vi "Cascade Config.vi"() -> (2 "FeedForward Constants Out":cluster{"kA":dbl, "kS":dbl, "kG":dbl, "kV":dbl}={"kA"=0.0, "kS"=0.0, "kG"=-0.25, "kV"=0.0}, 3 "Cascade Setpoints Config Out (Sensor Positions)":T2={"Array"=[{"Preset Name"=enum."Idle/Ground", "Cascade Pos"=0.0}, {"Preset Name"=enum."Raised L1", "Cascade Pos"=-3.112302245200002}, {"Preset Name"=enum."L2", "Cascade Pos"=-8.9212319508}, {"Preset Name"=enum."L2 Tip", "Cascade Pos"=-14.937623431600002}, {"Preset Name"=enum."L3", "Cascade Pos"=-21.991323788400003}, {"Preset Name"=enum."L3 Tip", "Cascade Pos"=-23.65101799}, {"Preset Name"=enum."Feeder", "Cascade Pos"=-16.4935867456}, {"Preset Name"=enum."\"Default\"", "Cascade Pos"=0.0}]})   [LabVIEW 2027]
uses:
  Cascade Positions.ctl
panel:
  in  "Cascade Setpoints Config (Sensor Pos)":T2={"Array"=[{"Preset Name"=enum."Idle/Ground", "Cascade Pos"=0.0}, {"Preset Name"=enum."Raised L1", "Cascade Pos"=8.0}, {"Preset Name"=enum."L2", "Cascade Pos"=15.0}, {"Preset Name"=enum."L2 Tip", "Cascade Pos"=16.0}, {"Preset Name"=enum."L3", "Cascade Pos"=20.0}, {"Preset Name"=enum."L3 Tip", "Cascade Pos"=22.0}, {"Preset Name"=enum."Feeder", "Cascade Pos"=13.0}, {"Preset Name"=enum."\"Default\"", "Cascade Pos"=0.0}]}
  in  "Cascade Setpoints Config (Inches of the Ground)":T2={"Array"=[{"Preset Name"=enum."Idle/Ground", "Cascade Pos"=21.25}, {"Preset Name"=enum."Raised L1", "Cascade Pos"=25.25}, {"Preset Name"=enum."L2", "Cascade Pos"=32.25}, {"Preset Name"=enum."L2 Tip", "Cascade Pos"=39.5}, {"Preset Name"=enum."L3", "Cascade Pos"=48.0}, {"Preset Name"=enum."L3 Tip", "Cascade Pos"=50.0}, {"Preset Name"=enum."Feeder", "Cascade Pos"=41.375}, {"Preset Name"=enum."\"Default\"", "Cascade Pos"=0.0}]}
  in  "FeedForward Constants In":cluster{"kA":dbl, "kS":dbl, "kG":dbl, "kV":dbl}={"kA"=0.0, "kS"=0.0, "kG"=0.18, "kV"=0.0}
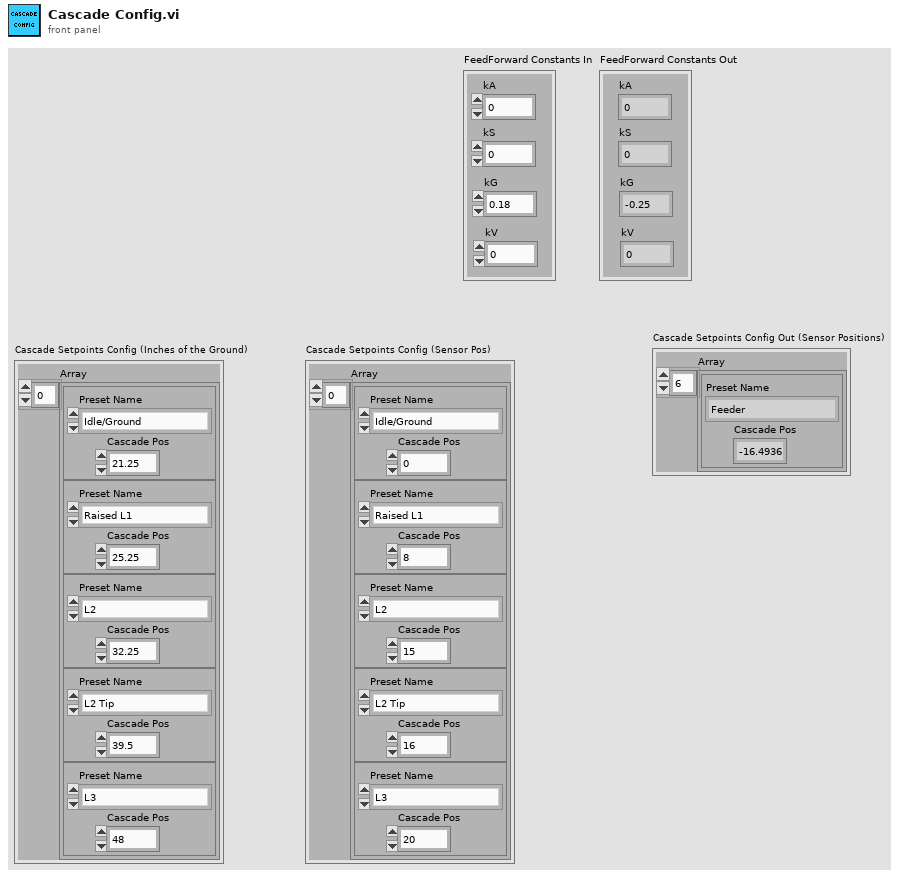
[diagram p1: front panel]
types:
  T1 = typedef "Cascade Positions.ctl" = enum16{"Idle/Ground", "Raised L1", "L2", "L2 Tip", "L3", "L3 Tip", "Feeder", "\"Default\""}
  T2 = cluster{"Array":cluster{"Preset Name":T1, "Cascade Pos":dbl}[]}
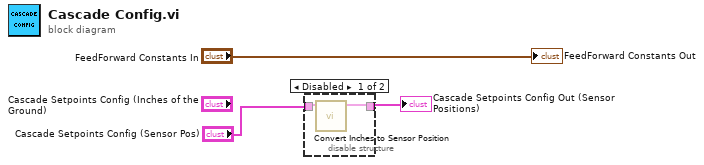
[diagram p0: block diagram]
diagram:
  n1 = disable-structure shown="Disabled" {
    disable-tunnel: "Cascade Setpoints Config (Sensor Pos)" -> [w5 w6]
    disable-tunnel: [w4 w6] -> w2
    frame Disabled {
      n2 = call "Convert Inches to Sensor Position.vi"("Cascade Setpoints Config in"=w5) -> ("Cluster"=w4:cluster{cluster{"Preset Name":T1, dbl}[]})  [unwired: 10 in]
    }
    frame Enabled {
    }
  }
  "Cascade Setpoints Config Out (Sensor Positions)" <- w2
  "FeedForward Constants Out" <- "FeedForward Constants In"
